vi "UI_Graph_Series.vi"(0 "Picture":picture, 1 "Y Min":dbl, 2 "Y Max":dbl=1.0, 5 "Samples":dbl[](array[numeric]), 7 "Color":u32, 9 "Plot Rect":T1={"left"=0, "top"=0, "right"=100, "bottom"=100}, 11 "error in":errorcluster) -> (4 "New Picture":picture, 15 "error out":errorcluster)   [LabVIEW 2026]
doc: "채널 1개 파형을 Plot Rect 안에 꺾은선으로 그린다(Y Min~Y Max)."
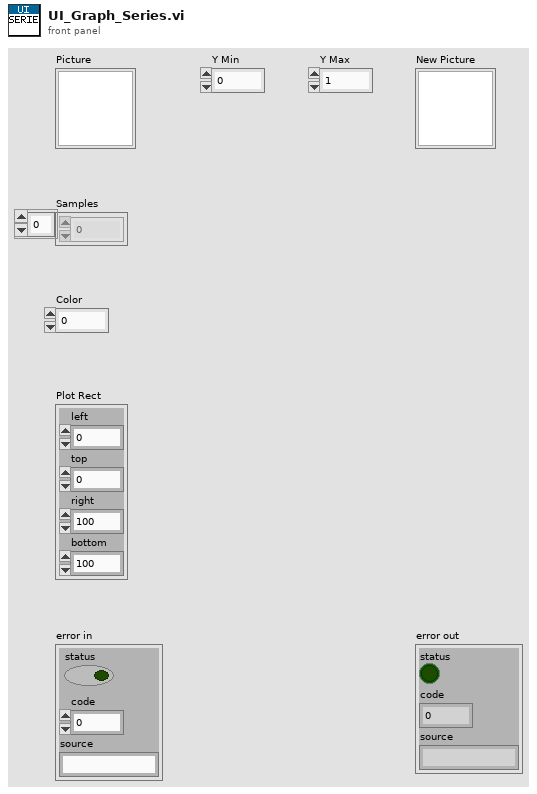
[diagram p1: front panel]
types:
  T1 = cluster{"left":i16, "top":i16, "right":i16, "bottom":i16}
  T2 = cluster{"Width":u16, "Style":enum32{"Solid", "Dash", "Dot", "DashDot", "DashDotDot"}}
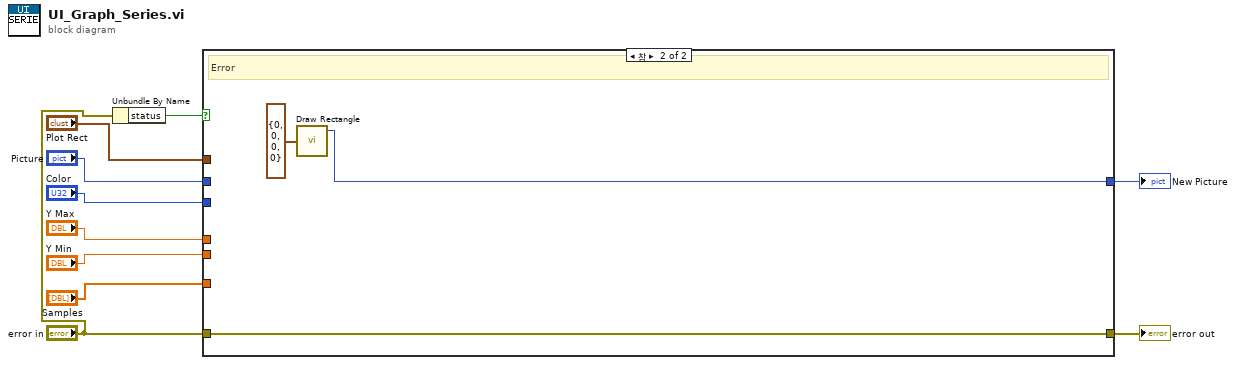
[diagram p0: block diagram]
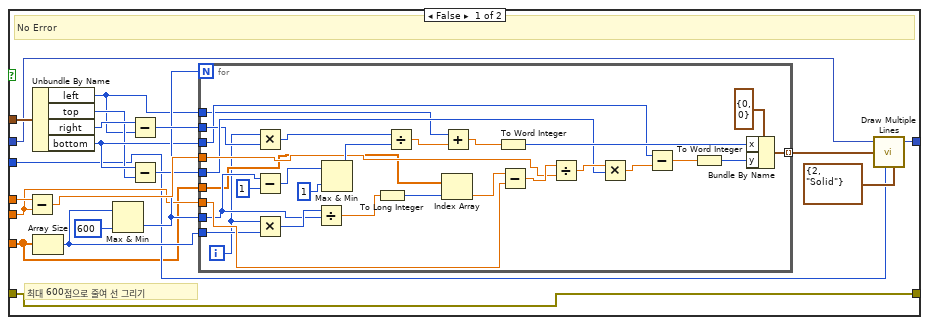
[diagram p2: hidden frame]
diagram:
  n1 = Unbundle By Name("error in") -> ("status"=w8:bool)
  n2 = case shown="참" w8 {
    tunnel: "Picture" -> [w11 _]
    tunnel: "Samples" -> [w12 _]
    tunnel: "Color" -> [w13 _]
    tunnel: "Plot Rect" -> [w14 _]
    tunnel: "Y Min" -> [w15 _]
    tunnel: "Y Max" -> [w16 _]
    tunnel: "error in" -> [w17 w60]
    tunnel: [w17 w60] -> w10
    tunnel: [w30 w62] -> w9
    frame False {
      # "최대 600점으로 줄여 선 그리기"
      # "No Error"
      n3 = Subtract(x=w16, y=w15) -> (x-y=w27:dbl)
      n4 = Unbundle By Name(w14) -> ("left"=w18:i16, "top"=w19:i16, "right"=w20:i16, "bottom"=w21:i16)
      n5 = Array Size(array=w12) -> (size(s)=w22:i32)
      n6 = Max & Min(x=w22, y=600) -> (min(x,y)=w24:i32)  [unwired: 1 out]
      n7 = Subtract(x=w20, y=w18) -> (x-y=w25:i16)
      n8 = Subtract(x=w21, y=w19) -> (x-y=w26:i16)
      n9 = for {
        N: w24 -> [_]
        tunnel: w12 -> [w32]
        tunnel: w15 -> [w39]
        tunnel: w22 -> [w33]
        tunnel: w18 -> [w35]
        tunnel: w21 -> [w36]
        tunnel: w27 -> [w40]
        tunnel: w24 -> [w34]
        tunnel: w25 -> [w37]
        tunnel: w26 -> [w38]
        tunnel: [w59] -> w28 mode=indexing
        i -> [w31]
        n10 = Multiply(x=w31, y=w37) -> (x*y=w49:i32)
        n11 = Subtract(x=w34, y=1) -> (x-y=w46:i32)
        n12 = Multiply(x=w31, y=w33) -> (x*y=w41:i32)
        n13 = Divide(x=w41, y=w34) -> (x/y=w42:dbl)
        n14 = Max & Min(x=w46, y=1) -> (max(x,y)=w48:i32)  [unwired: 1 out]
        n15 = To Long Integer(number=w42) -> (32bit integer=w43:i32)
        n16 = Divide(x=w49, y=w48) -> (x/y=w50:dbl)
        n17 = Index Array(array=w32, index=w43) -> (element=w44:dbl)
        n18 = Add(x=w35, y=w50) -> (x+y=w51:dbl)
        n19 = To Word Integer(number=w51) -> (16bit integer=w57:i16)
        n20 = Subtract(x=w44, y=w39) -> (x-y=w52:dbl)
        n21 = Divide(x=w52, y=w40) -> (x/y=w53:dbl)
        n22 = Multiply(x=w53, y=w38) -> (x*y=w54:dbl)
        n23 = Subtract(x=w36, y=w54) -> (x-y=w55:dbl)
        n24 = To Word Integer(number=w55) -> (16bit integer=w58:i16)
        n25 = Bundle By Name(cluster=cluster{"x":i16, "y":i16} {"x"=0, "y"=0}, "x"=w57, "y"=w58) -> (w59:cluster{"x":i16, "y":i16})
      }
      n26 = call <vilib>:"Draw Multiple Lines.vi"("picture"=w11, "line endpoints"=w28, "color(black)"=w13, "pen"=T2 {"Width"=2, "Style"=enum."Solid"}) -> ("new picture"=w30:picture)  [unwired: 5 in]
    }
    frame True {
      # "Error"
      n27 = call <vilib>:"Draw Rectangle.vi"("rect"=T1 {"left"=0, "top"=0, "right"=0, "bottom"=0}) -> ("new picture"=w62:picture)  [unwired: 8 in]
    }
  }
  "New Picture" <- w9
  "error out" <- w10
